vi "Push.vi"(6 "Route":string, 8 "error in (no error)":errorcluster, 11 "Navigator in":refnum<class "Navigator.lvclass">) -> (0 "error out":errorcluster, 3 "Navigator out":refnum<class "Navigator.lvclass">)   [LabVIEW 2024, in "Navigator.lvclass"]
doc: "Push route onto Navigator stack."
uses:
  Navigator.lvclass
  Navigator.lvclass/Navigator.ctl
  NavigatableView/NavigatableView.lvclass
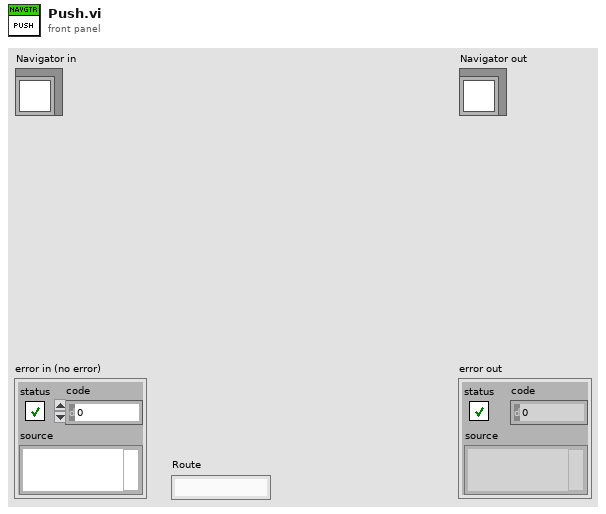
[diagram p1: front panel]
types:
  T1 = typedef "Navigator.lvclass/Route.ctl" = cluster{"Name":string, "Path":path, "Builder":refnum<class "NavigatableView.lvclass">}
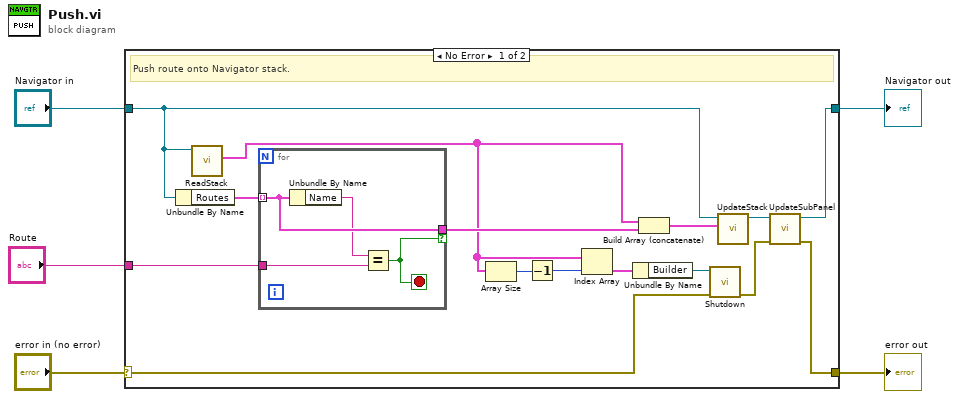
[diagram p0: block diagram]
diagram:
  n1 = case shown="No Error" "error in (no error)" {
    selector: "error in (no error)" -> [w12 w26]
    tunnel: [w13 w26] -> w2
    tunnel: [w14 w25] -> w3
    tunnel: "Navigator in" -> [w7 w25]
    tunnel: "Route" -> [w18 _]
    frame No Error {
      # "Push route onto Navigator stack."
      n2 = Unbundle By Name(w7) -> ("Routes"=w20:T1[])
      n3 = call "ReadStack.vi"("Navigator in"=w7) -> ("Stack"=w9:T1[])  [unwired: 8 in, 2 out]
      n4 = for {
        tunnel: w20 -> [w24] mode=indexing
        tunnel: [w24] -> w19 if=w22
        tunnel: w18 -> [w21]
        stop <- w22 stop-if-true
        n5 = Unbundle By Name(w24) -> ("Name"=w23:string)
        n6 = Equal?(x=w23, y=w21) -> (x = y?=w22:bool)
      }
      n7 = Array Size(array=w9) -> (size(s)=w17:i32)
      n8 = Decrement(x=w17) -> (x-1=w16:i32)
      n9 = Index Array(array=w9, index=w16) -> (element=w15:T1)
      n10 = Unbundle By Name(w15) -> ("Builder"=w10:refnum<class "NavigatableView.lvclass">)
      n11 = Build Array (concatenate)(w9, w19) -> (w8:T1[])
      n12 = call-dynamic "Shutdown.vi"("error in (no error)"=w12, "NavigatableView in"=w10) -> ("error out"=w11:errorcluster)  [unwired: 8 in, 1 out]
      n13 = call "UpdateStack.vi"("Stack"=w8, "Navigator in"=w7) -> ("Navigator out"=w6:refnum<class "Navigator.lvclass">)  [unwired: 8 in, 1 out]
      n14 = call "UpdateSubPanel.vi"("error in (no error)"=w11, "Navigator in"=w6) -> ("error out"=w13:errorcluster, "Navigator out"=w14:refnum<class "Navigator.lvclass">)  [unwired: 8 in]
    }
    frame Error {
    }
  }
  "error out" <- w2
  "Navigator out" <- w3
